vi "AlliGator Panel Paths.vi"(8 "Error In":errorcluster, 11 "Application Directory":path) -> (0 "Error Out":errorcluster, 3 "SubPanel VI Paths in AlliGator Folder":path[](array[path]))   [LabVIEW 2021, in "AlliGator GUI.lvlib"]
uses:
  AlliGator GUI.lvlib
  <userlib>/_OpenG.lib/file/file.llb/Compare Two Paths - Scalar__ogtk.vi
  <userlib>/_OpenG.lib/file/file.llb/openg_file.lvlib
panel:
  in  "Panel Paths":string[](array[string])
  # "Save this array of relative paths as constant on BD before creating a standalone application"
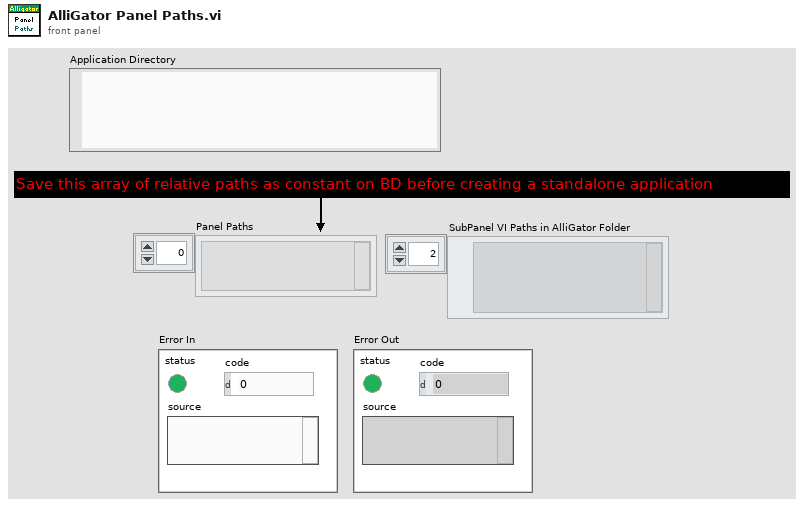
[diagram p1: front panel]
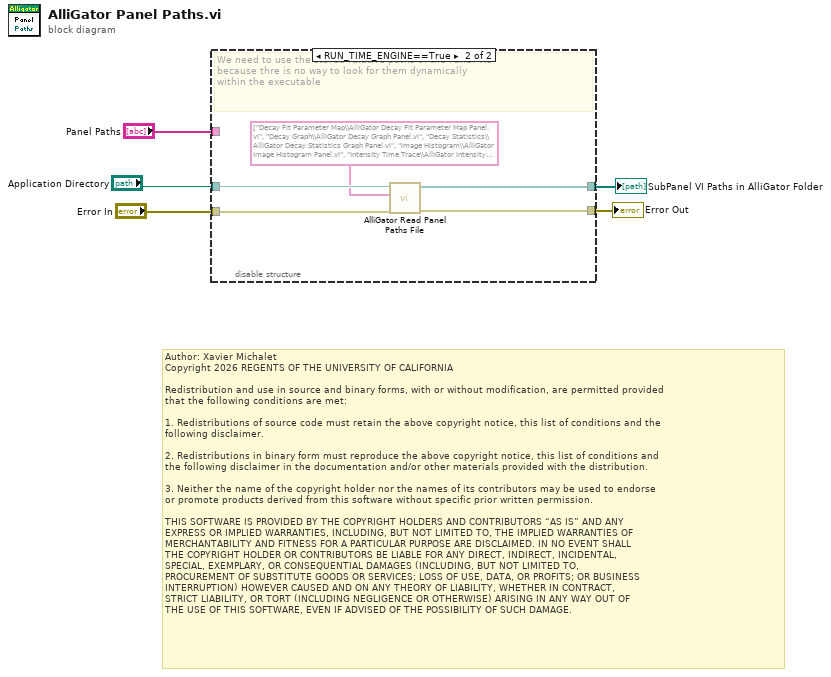
[diagram p0: block diagram]
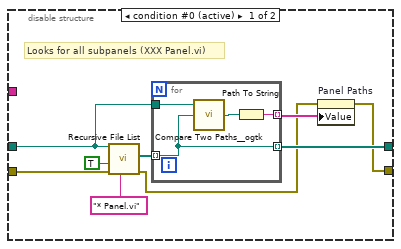
[diagram p2: hidden frame]
diagram:
  # "Author: Xavier Michalet\nCopyright 2026 REGENTS OF THE UNIVERSITY OF CALIFORNIA\n\nRedistribution and use in source and binary forms, with or without modification, are permitted provided\nthat the following conditions are met:\n\n1. Redistributions of source code must retain the above copyright notice, this list of conditions and the\nfollowing disclaimer.\n\n2. Redistributions in binary form must reproduce the above copyright notice, this list of conditions and\nthe following disclaimer in the documentation and/or other materials provided with the distribution.\n\n3. Neither the name of the copyright holder nor the names of its contributors may be used to endorse \nor promote products derived from this software without specific prior written permission.\n\nTHIS SOFTWARE IS PROVIDED BY THE COPYRIGHT HOLDERS AND CONTRIBUTORS “AS IS” AND ANY \nEXPRESS OR IMPLIED WARRANTIES, INCLUDING, BUT NOT LIMITED TO, THE IMPLIED WARRANTIES OF\nMERCHANTABILITY AND FITNESS FOR A PARTICULAR PURPOSE ARE DISCLAIMED. IN NO EVENT SHALL\nTHE COPYRIGHT HOLDER OR CONTRIBUTORS BE LIABLE FOR ANY DIRECT, INDIRECT, INCIDENTAL, \nSPECIAL, EXEMPLARY, OR CONSEQUENTIAL DAMAGES (INCLUDING, BUT NOT LIMITED TO, \nPROCUREMENT OF SUBSTITUTE GOODS OR SERVICES; LOSS OF USE, DATA, OR PROFITS; OR BUSINESS\nINTERRUPTION) HOWEVER CAUSED AND ON ANY THEORY OF LIABILITY, WHETHER IN CONTRACT, \nSTRICT LIABILITY, OR TORT (INCLUDING NEGLIGENCE OR OTHERWISE) ARISING IN ANY WAY OUT OF\nTHE USE OF THIS SOFTWARE, EVEN IF ADVISED OF THE POSSIBILITY OF SUCH DAMAGE."
  n1 = disable-structure shown="RUN_TIME_ENGINE==True" {
    disable-tunnel: [w11 w22] -> w5
    disable-tunnel: "Error In" -> [w10 w23]
    disable-tunnel: [w6 w21] -> w3
    disable-tunnel: "Application Directory" -> [w9 w20]
    disable-tunnel: "Panel Paths" -> [_ _]
    frame condition #0 (active) {
      # "Looks for all subpanels (XXX Panel.vi)"
      n2 = call <vilib>:"Recursive File List.vi"("pattern"="* Panel.vi", "error in (no error)"=w10, "Continue Recursing on Error? (F)"=TRUE, "Folder Path"=w9) -> ("error out"=w7:errorcluster, "All Files in Dir"=w12:path[])  [unwired: 3 in, 3 out]
      n3 = for {
        tunnel: w12 -> [w15] mode=indexing
        tunnel: w9 -> [w18]
        tunnel: [w15] -> w11 mode=indexing
        tunnel: [w16] -> w8 mode=indexing
        n4 = call-poly <userlib>:"Compare Two Paths__ogtk.vi"("path2"=w15, "path1"=w18) -> ("relative path from 1 to 2"=w17:path)  [unwired: 1 in, 2 out]
        n5 = Path To String(path=w17) -> (string=w16:string)
      }
      n6 = property on="Panel Paths" class="Arr (strict)"(error in=w7, "Value"=w8) -> (error out=w6:errorcluster)  [unwired: 1 in, 1 out]
    }
    frame condition #1 {
      # "We need to use the stored relative paths of the Panel VIs\nbecause thre is no way to look for them dynamically\nwithin the executable"
      n7 = call "AlliGator Read Panel Paths File.vi"("error in (no error)"=w23, "Panel File Paths"=string[] ["Decay Fit Parameter Map\\AlliGator Decay Fit Parameter Map Panel.vi", "Decay Graph\\AlliGator Decay Graph Panel.vi", "Decay Statistics\\AlliGator Decay Statistics Graph Panel.vi", "Image Histogram\\AlliGator Image Histogram Panel.vi", "Intensity Time Trace\\AlliGator Intensity Time Trace Panel.vi", "Lifetime & Other Parameters\\AlliGator Lifetime & Other Parameters Panel.vi", "Parameter Map\\AlliGator Parameter Map Panel.vi", "Phasor Graph\\AlliGator Phasor Graph Panel.vi", "Phasor Plot\\AlliGator Phasor Plot Panel.vi", "Phasor Ratio\\AlliGator Phasor Ratio Graph Panel.vi"] ("Panel Paths"), "Application Directory"=w20) -> ("error out"=w21:errorcluster, "Panel File Paths"=w22:path[])  [unwired: 7 in]
    }
  }
  "SubPanel VI Paths in AlliGator Folder" <- w5
  "Error Out" <- w3
